vi "clone.vi"(0 "reference":refnum<class "ClassRelationshipEdge.lvclass">, 5 "error in (no error)":errorcluster) -> (14 "reference out":refnum<class "ClassRelationshipEdge.lvclass">, 15 "clonedEdge":refnum<class "AbstractEdge.lvclass">, 19 "error out":errorcluster)   [LabVIEW 2020, in "ClassRelationshipEdge.lvclass"]
uses:
  <resource>/Framework/Providers/Open_GDS/UML/ClassRelationshipEdge_class/ClassRelationshipEdge.lvclass
  C:/Program Files (x86)/National Instruments/LabVIEW 2020/resource/Framework/Providers/Open_GDS/UML/SegmentedLineEdge_class/SegmentedLineEdge.lvclass
  C:/Program Files (x86)/National Instruments/LabVIEW 2020/resource/Framework/Providers/Open_GDS/UML/GeneralPathEdge_class/GeneralPathEdge.lvclass
  C:/Program Files (x86)/National Instruments/LabVIEW 2020/resource/Framework/Providers/Open_GDS/UML/AbstractEdge_class/AbstractEdge.lvclass
  <resource>/Framework/Providers/Open_GDS/UML/AbstractEdge_class/AbstractEdge.lvclass
  <resource>/Framework/Providers/Open_GDS/UML/SegmentedLineEdge_class/SegmentedLineEdge.lvclass
  <resource>/Framework/Providers/Open_GDS/UML/GeneralPathEdge_class/GeneralPathEdge.lvclass
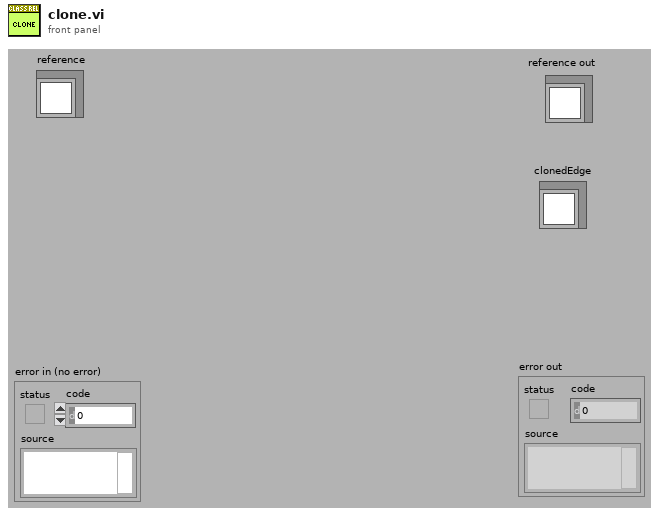
[diagram p1: front panel]
types:
  T1 = typedef "ClassRelationshipEdge.lvclass/ObjectAttributes.ctl" = cluster{"bentStyleRef":refnum<class "BentStyle.lvclass">, "startConnectionOffset":cluster{"x":i32, "y":i32}, "endConnectionOffset":cluster{"x":i32, "y":i32}, "MidLineOffset":cluster{"x":i32, "y":i32}, "DepClass":T2}
  T2 = typedef "ReversedEngineering_ViDependencyDetailsType.ctl" = cluster{"ThisVIs/Ctls":path[], "Dependent_VIs/Ctls":path[]}
  T3 = typedef "SegmentedLineEdge.lvclass/ObjectAttributes.ctl" = cluster{"lineStyle":refnum<class "LineStyle.lvclass">, "startArrowHead":refnum<class "ArrowHead.lvclass">, "endArrowHead":refnum<class "ArrowHead.lvclass">, "startLabel":string, "midLabel":string, "endLabel":string, "MidLabelOffset":T4, "SplitWire":bool}
  T4 = typedef "Point Point2D.ctl" = cluster{"x":dbl, "y":dbl}
  T5 = typedef "GeneralPathEdge.lvclass/ObjectAttributes.ctl" = cluster{"None":bool}
  T6 = typedef "AbstractEdge.lvclass/ObjectAttributes.ctl" = cluster{"start":refnum<class "AbstractNode.lvclass">, "end":refnum<class "AbstractNode.lvclass">}
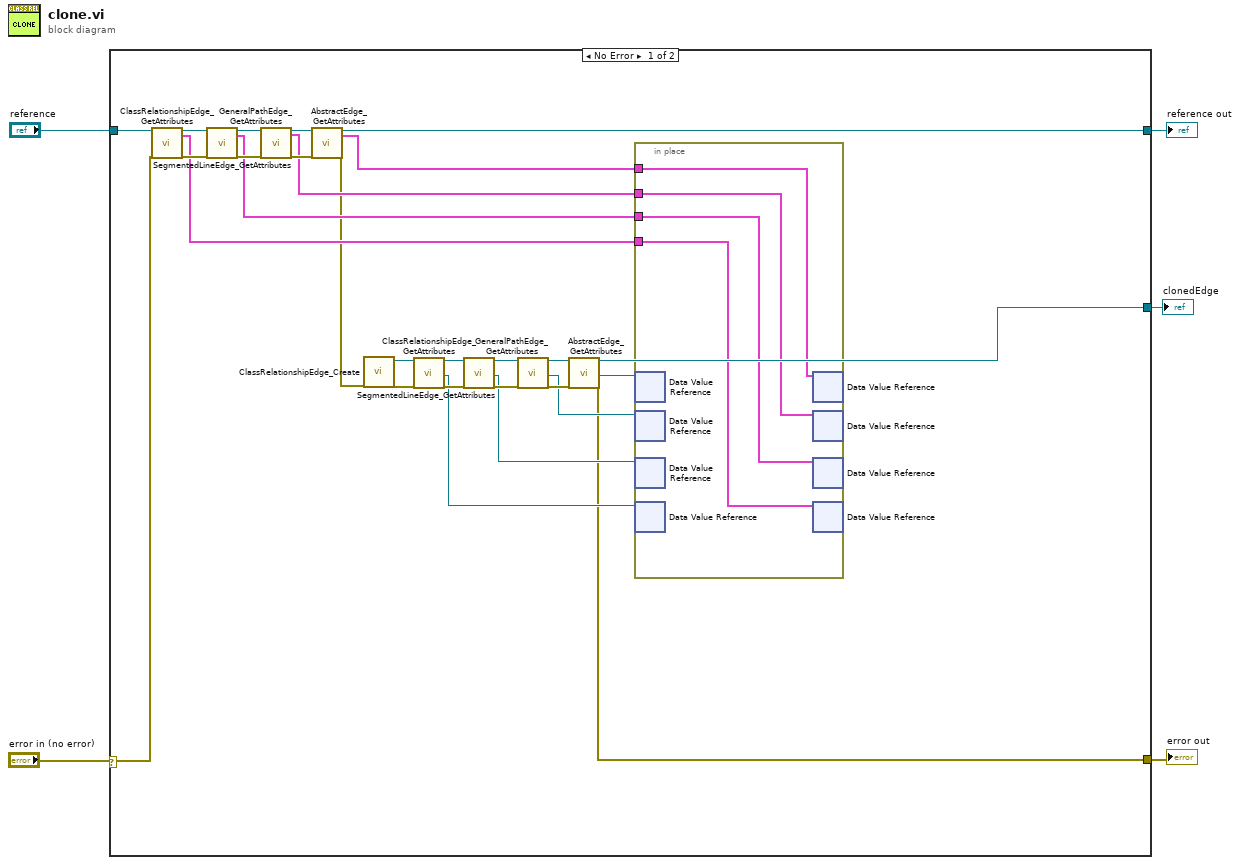
[diagram p0: block diagram]
diagram:
  n1 = case shown="No Error" "error in (no error)" {
    selector: "error in (no error)" -> [w11 w38]
    tunnel: "reference" -> [w10 w39]
    tunnel: [w7 w38] -> w4
    tunnel: [w9 w39] -> w3
    tunnel: [w8 _] -> w1
    frame No Error {
      n2 = call <resource>:"ClassRelationshipEdge_GetAttributes.vi"("reference in"=w10, "error in (no error)"=w11) -> ("reference out"=w33:refnum<class "ClassRelationshipEdge.lvclass">, "Data"=w21:T1, "error out"=w32:errorcluster)  [unwired: 1 in, 14 out]
      n3 = call <resource>:"SegmentedLineEdge_GetAttributes.vi"("reference in"=w33, "error in (no error)"=w32) -> ("reference out"=w29:refnum<class "ClassRelationshipEdge.lvclass">, "Data"=w20:T3, "error out"=w28:errorcluster)  [unwired: 1 in, 14 out]
      n4 = call <resource>:"GeneralPathEdge_GetAttributes.vi"("reference in"=w29, "error in (no error)"=w28) -> ("reference out"=w31:refnum<class "ClassRelationshipEdge.lvclass">, "Data"=w19:T5, "error out"=w30:errorcluster)  [unwired: 14 in, 1 out]
      n5 = call <resource>:"AbstractEdge_GetAttributes.vi"("reference in"=w31, "error in (no error)"=w30) -> ("reference out"=w9:refnum<class "ClassRelationshipEdge.lvclass">, "Data"=w18:T6, "error out"=w6:errorcluster)  [unwired: 14 in, 1 out]
      n6 = call <resource>:"ClassRelationshipEdge_Create.vi"("error in (no error)"=w6) -> ("reference out"=w13:refnum<class "ClassRelationshipEdge.lvclass">, "error out"=w12:errorcluster)  [unwired: 17 in]
      n7 = call <resource>:"ClassRelationshipEdge_GetAttributes.vi"("reference in"=w13, "error in (no error)"=w12) -> ("reference out"=w23:refnum<class "ClassRelationshipEdge.lvclass">, "DataRef"=w15:refnum<data-value>, "error out"=w22:errorcluster)  [unwired: 1 in, 14 out]
      n8 = call <resource>:"SegmentedLineEdge_GetAttributes.vi"("reference in"=w23, "error in (no error)"=w22) -> ("reference out"=w26:refnum<class "ClassRelationshipEdge.lvclass">, "DataRef"=w16:refnum<data-value>, "error out"=w27:errorcluster)  [unwired: 1 in, 14 out]
      n9 = call <resource>:"GeneralPathEdge_GetAttributes.vi"("reference in"=w26, "error in (no error)"=w27) -> ("reference out"=w24:refnum<class "ClassRelationshipEdge.lvclass">, "DataRef"=w14:refnum<data-value>, "error out"=w25:errorcluster)  [unwired: 14 in, 1 out]
      n10 = call <resource>:"AbstractEdge_GetAttributes.vi"("reference in"=w24, "error in (no error)"=w25) -> ("reference out"=w8:refnum<class "ClassRelationshipEdge.lvclass">, "DataRef"=w17:refnum<data-value>, "error out"=w7:errorcluster)  [unwired: 14 in, 1 out]
      n11 = in-place {
        in-place-border: w21 -> [w37]
        in-place-border: w20 -> [w36]
        in-place-border: w19 -> [w35]
        in-place-border: w18 -> [w34]
        n12 = in-place-dvr #1(w17) -> ()  [unwired: 2 out]
        n13 = in-place-dvr #2(w14) -> ()  [unwired: 2 out]
        n14 = in-place-dvr #3(w16) -> ()  [unwired: 2 out]
        n15 = in-place-dvr #4(w15) -> ()  [unwired: 2 out]
        n16 = in-place-dvr #1(w34) -> ()  [unwired: 2 out]
        n17 = in-place-dvr #2(w35) -> ()  [unwired: 2 out]
        n18 = in-place-dvr #3(w36) -> ()  [unwired: 2 out]
        n19 = in-place-dvr #4(w37) -> ()  [unwired: 2 out]
      }
    }
    frame Error {
    }
  }
  "reference out" <- w3
  "error out" <- w4
  "clonedEdge" <- w1
